vi "Test_pgADONet_dist.vi"() -> ()   [LabVIEW 2026]
uses:
  <vilib>/Viviota/shared/ORM.lvlibp/TypeMap/TypeMap.lvclass
  <vilib>/Viviota/shared/ORM_lib.lvlibp/ObjectRow/ObjectLUT.lvclass
  <vilib>/numeric/Random Number (Range) I64.vi
  <vilib>/numeric/Random Number (Range) DBL.vi
  f3693442-7653-4e44-a421-498bef5f0c13.vi
  <vilib>/Analysis/baseanly.llb/Mean (DBL).vi
  <vilib>/numeric/sub_Random U32.vi
  <vilib>/Viviota/shared/ORM_ADONet.lvlibp/ADOMapper/ADOMapper.lvclass
  C:/Program Files/National Instruments/LabVIEW 2026/vi.lib/Viviota/shared/ORM.lvlibp/SqlMapper/SqlMapper.lvclass
  <vilib>/JDP Science/JSONtext/Variant to JSON Text.vi
  <vilib>/Viviota/shared/ORM_lib.lvlibp/ObjectRow/Write LUT.vi
  <vilib>/Viviota/shared/ORM_DBC_Npgsql_netCore.lvlibp/Postgresql Connect.vi
  <vilib>/Viviota/shared/ORM_pgsql_jdp.lvlibp/dbc/Postgresql Connect.vi
  <vilib>/Viviota/shared/ORM_DBC_Npgsql.lvlibp/Postgresql Connect.vi
  <vilib>/Viviota/shared/ORM.lvlibp/SqlMapper/Read DbConnection.vi
  <vilib>/Viviota/shared/ORM.lvlibp/DbConnection/Write SupportTX.vi
  <vilib>/Viviota/shared/ORM.lvlibp/SqlMapper/Write DbConnection.vi
  <vilib>/Viviota/shared/ORM.lvlibp/TypeMap/Write Table Name.vi
  <vilib>/Viviota/shared/ORM.lvlibp/TypeMap/Write Autokey.vi
  <vilib>/Viviota/shared/ORM_lib.lvlibp/ObjectRow/Read LUT.vi
  <vilib>/JDP Science/JSONtext/LVClass Serializer/JSONtext LVClass Serializer.lvclass
  <vilib>/Viviota/shared/ORM_ADONetCore.lvlibp/ADOMapper/ADOMapper.lvclass
  <vilib>/Viviota/shared/ORM.lvlibp/DbConnection/DbConnection.lvclass
  <vilib>/Viviota/shared/ORM.lvlibp/SqlMapper/SqlMapper.lvclass
  C:/Program Files/National Instruments/LabVIEW 2026/vi.lib/Viviota/shared/ORM_ADONetCore.lvlibp/ADOMapper/ADOMapper.lvclass
  C:/Program Files/National Instruments/LabVIEW 2026/vi.lib/Viviota/shared/ORM_ADONet.lvlibp/ADOMapper/ADOMapper.lvclass
  <vilib>/Analysis/NI_AALBase.lvlib
  <vilib>/Viviota/Viviota ORM - NetCore Connections/dotNetCore/NetCore_API/ORM_API_NetCore.lvlib
  <vilib>/Viviota/Viviota ORM - Direct Connections/DirectConnections/API/ORM_API_jdp.lvlib
  <vilib>/Viviota/Viviota ORM/ORM_API/ORM_API.lvlib
  <vilib>/Viviota/shared/ORM_DBC_Npgsql_netCore.lvlibp/DBC.lvclass
  <vilib>/Viviota/shared/ORM_pgsql_jdp.lvlibp/dbc/DBC.lvclass
  <vilib>/Viviota/shared/ORM_DBC_Npgsql.lvlibp/DBC.lvclass
panel:
  out "Numeric 2":i32
  out "Numeric":i32
  out "mean 3":dbl format="%0.6f"
  out "mean 2":dbl format="%0.6f"
  out "mean":dbl format="%0.6f"
  out "x-y":dbl[](array[numeric])
  out "Array 2":dbl[](array[numeric])
  out "Array":dbl[](array[numeric])
  out "LUT 2":variant[](array[variant])
  out "LUT":variant[](array[variant])
  out "id":i32[](array[numeric])
  # "0.016\n0.084\n0.040"
  # "0.0171\n0.00513\n0.00119"
  # "0.0187\n0.0159\n0.0041"
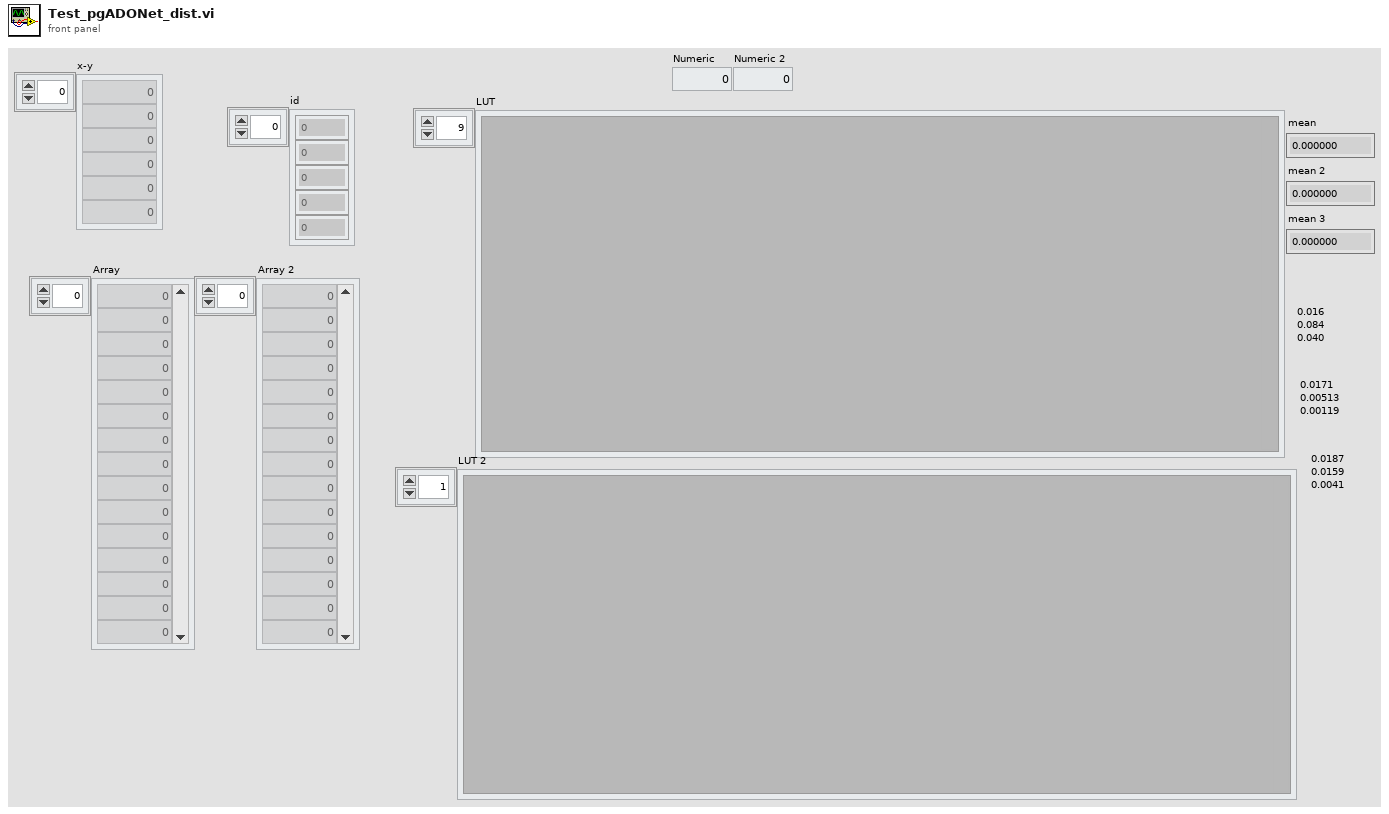
[diagram p1: front panel]
types:
  T1 = cluster{"Text":string, "Integer":i32, "dbl":dbl, "timestamp":timestamp}
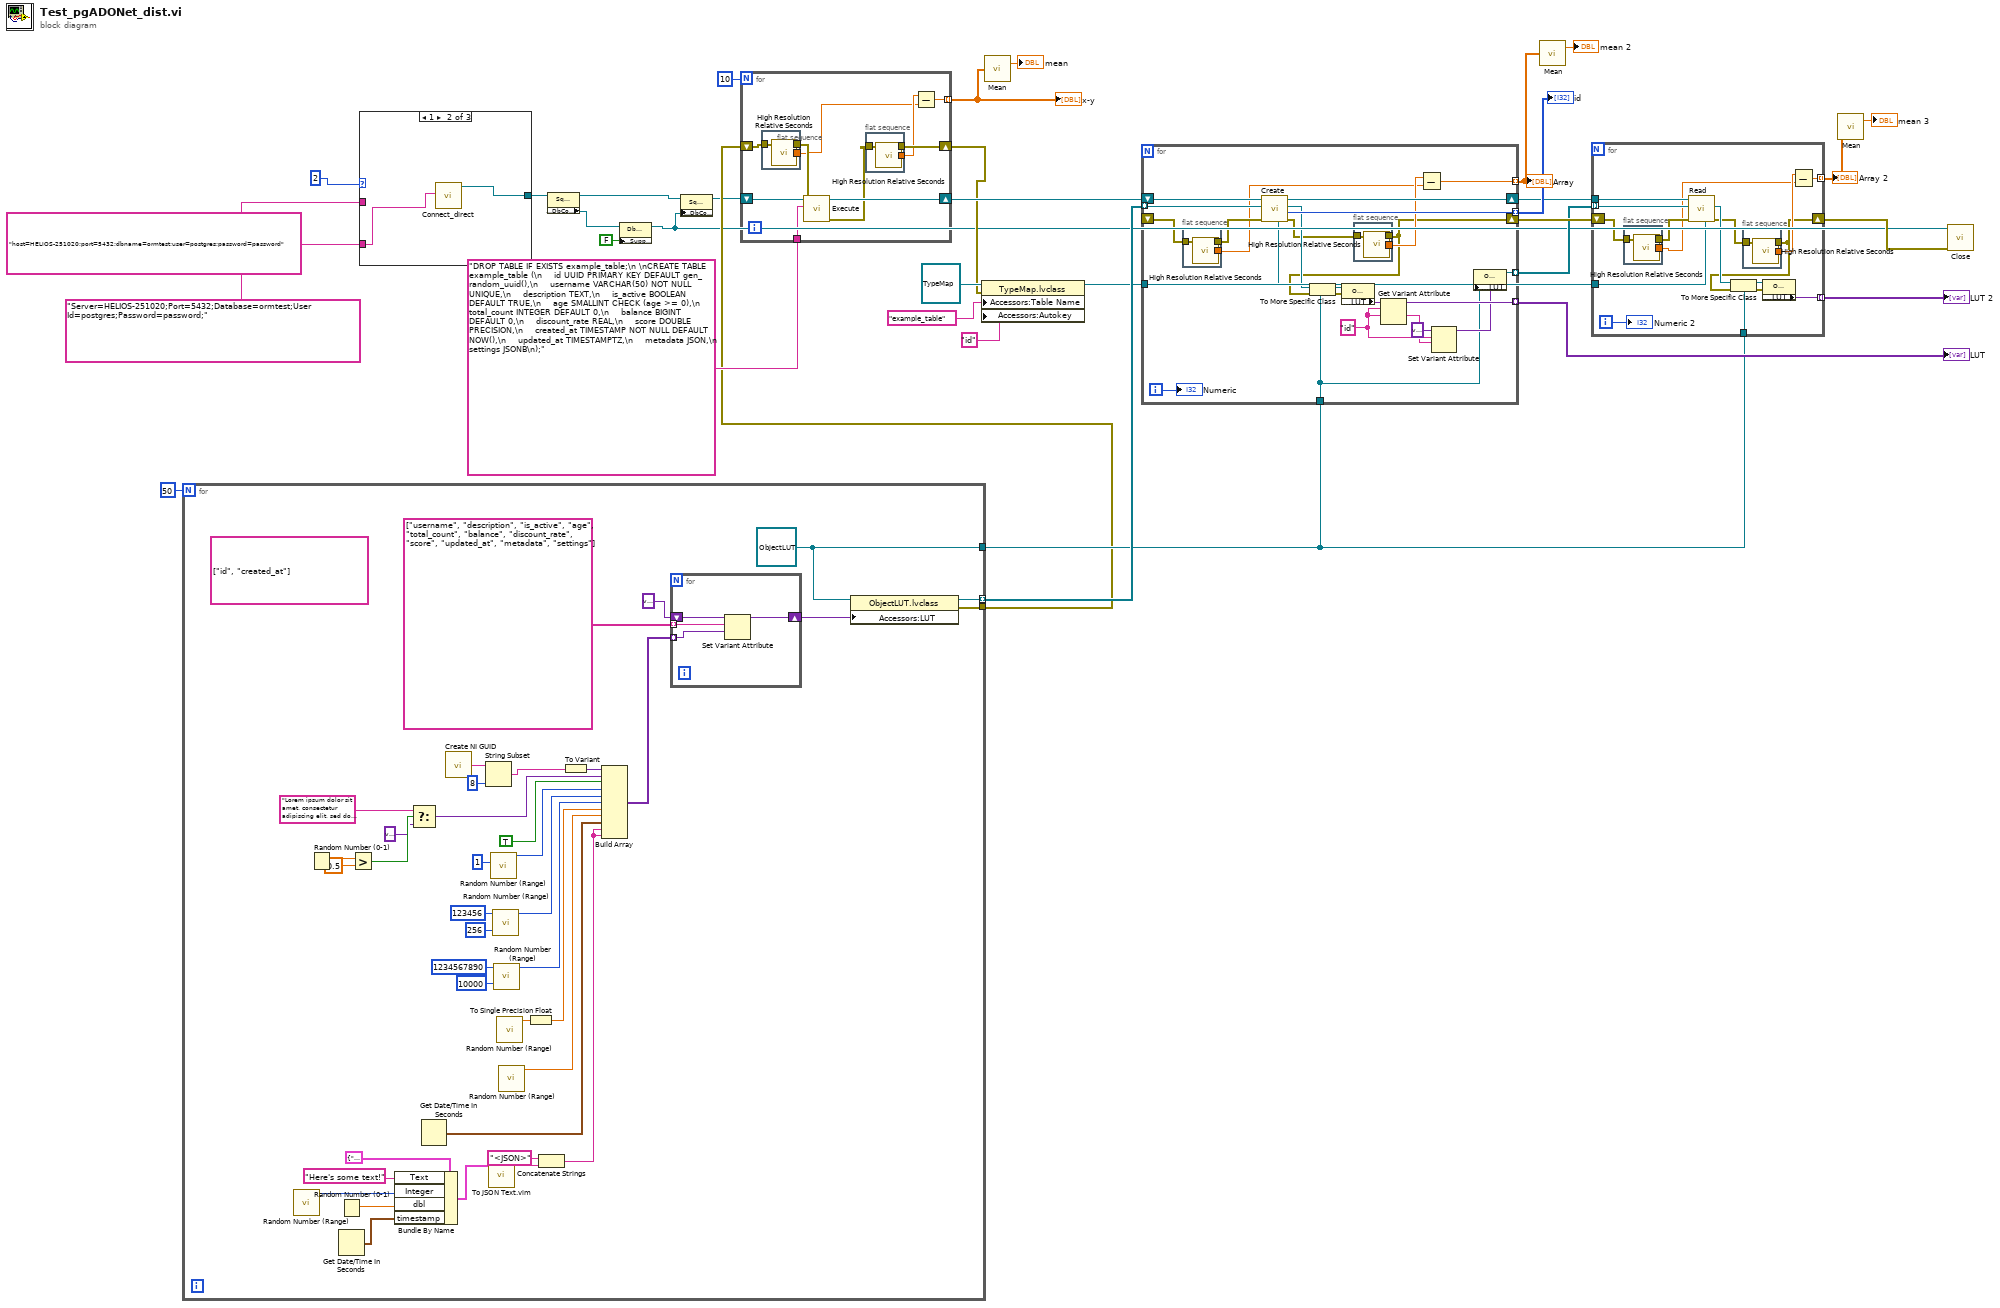
[diagram p0: block diagram]
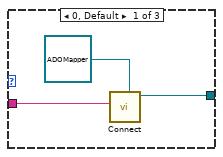
[diagram p2: hidden frame]
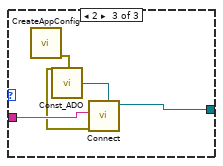
[diagram p3: hidden frame]
diagram:
  n1 = for {
    N: 50 -> [_]
    tunnel: [w41] -> w33 mode=indexing
    tunnel: [w40] -> w23
    tunnel: [w35] -> w18
    w40 = refnum<class "ObjectLUT.lvclass"> refnum ("ORM_lib.lvlibp:ObjectLUT.lvclass")
    (unwired) string[] ["id", "created_at"]
    n2 = call-poly <vilib>:"Random Number (Range).vi"() -> ("number"=w48:i64)  [unwired: 11 in]
    n3 = Random Number (0-1)() -> (number: 0 to 1=w57:dbl)
    n4 = Random Number (0-1)() -> (number: 0 to 1=w49:dbl)
    n5 = Get Date/Time In Seconds() -> (seconds since 1Jan1904=w50:timestamp)
    n6 = Greater?(x=w57, y=0.5) -> (0:w55:bool)
    n7 = Bundle By Name(cluster=T1 {"Text"="This is a test", "Integer"=0, "dbl"=0.0, "timestamp"=timestamp(0 s since 1904-01-01)}, "Text"="Here's some text!", "Integer"=w48, "dbl"=w49, "timestamp"=w50) -> (w46:T1)
    n8 = Select(t="Lorem ipsum dolor sit amet, consectetur adipiscing elit, sed do eiusmod tempor incididunt ut labore et dolore magna aliqua", s=w55, f=variant) -> (s? t:f=w53:variant)
    n9 = Get Date/Time In Seconds() -> (seconds since 1Jan1904=w47:timestamp)
    n10 = call <vilib>:"Create NI GUID.vi"() -> ("NI GUID"=w73:string)
    n11 = String Subset(string=w73, length (rest)=8 ("length (rest)")) -> (substring=w68:string)  [unwired: 1 in]
    n12 = call "To JSON Text.vim"("Anything"=w46) -> ("<JSON>"=w39:string)  [unwired: 9 in, 1 out]
    n13 = call-poly <vilib>:"Random Number (Range).vi"("lower bound (-100)"=i64 1) -> ("number"=w65:i64)  [unwired: 10 in]
    n14 = call-poly <vilib>:"Random Number (Range).vi"("lower bound (-100)"=i64 256, "upper bound (100)"=i64 123456) -> ("number"=w64:i64)  [unwired: 9 in]
    n15 = call-poly <vilib>:"Random Number (Range).vi"("lower bound (-100)"=i64 10000, "upper bound (100)"=i64 1234567890) -> ("number"=w63:i64)  [unwired: 9 in]
    n16 = call-poly <vilib>:"Random Number (Range).vi"() -> ("number"=w61:dbl)  [unwired: 11 in]
    n17 = call-poly <vilib>:"Random Number (Range).vi"() -> ("number"=w59:dbl)  [unwired: 11 in]
    n18 = To Single Precision Float(number=w61) -> (single precision float=w60:sgl)
    n19 = Concatenate Strings("<JSON>" ("string"), w39) -> (w38:string)
    n20 = To Variant(anything=w68) -> (Variant=w67:variant)
    n21 = Build Array(w67, w53, TRUE, w65, w64, w63, w60, w59, w47, w38, w38) -> (w44:variant[])
    n22 = for {
      tunnel: string[] ["username", "description", "is_active", "age", "total_count", "balance", "discount_rate", "score", "updated_at", "metadata", "settings"] -> [w77] mode=indexing
      tunnel: w44 -> [w76] mode=indexing
      shift-right: [w75] -> w42
      shift-left: variant -> [w74]
      n23 = Set Variant Attribute(Variant=w74, name=w77, value=w76) -> (Variant out=w75:variant)  [unwired: 1 in, 2 out]
    }
    n24 = property class="ObjectLUT.lvclass"(reference=w40, "Accessors:LUT"=w42) -> (reference out=w41:refnum<class "ObjectLUT.lvclass">, error out=w35:errorcluster)  [unwired: 1 in]
  }
  n25 = case shown="1" 2 {
    tunnel: "Server=HELIOS-251020;Port=5432;Database=ormtest;User Id=postgres;Password=password;" ("Connection String") -> [w80 _ w84]
    tunnel: [w78 w82 w86] -> w8
    tunnel: "host=HELIOS-251020;port=5432;dbname=ormtest;user=postgres;password=password" ("Connection String") -> [_ w81 _]
    frame 0, Default {
      n26 = call-poly <vilib>:"Connect.vi"("SqlMapper Type"=refnum<class "ADOMapper.lvclass"> refnum ("ORM_ADONetCore.lvlibp:ADOMapper.lvclass"), "Connection String"=w80) -> ("SqlMapper out"=w78:refnum<class "ADOMapper.lvclass">)  [unwired: 8 in, 1 out]
    }
    frame 1 {
      n27 = call-poly <vilib>:"Connect_direct.vi"("Connection String"=w81) -> ("SqlMapper out"=w82:refnum<class "SqlMapper.lvclass">)  [unwired: 9 in, 1 out]
    }
    frame 2 {
      n28 = call <vilib>:"CreateAppConfig.vi"() -> ("error out"=w83:errorcluster)  [unwired: 11 in]
      n29 = call <vilib>:"Const_ADO.vi"() -> ("ADOMapper"=w85:refnum<class "ADOMapper.lvclass">)
      n30 = call-poly <vilib>:"Connect.vi"("SqlMapper Type"=w85, "error in (no error)"=w83, "Connection String"=w84) -> ("SqlMapper out"=w86:refnum<class "ADOMapper.lvclass">)  [unwired: 7 in, 1 out]
    }
  }
  n31 = property class="SqlMapper.lvclass"(reference=w8) -> (reference out=w5:refnum<class "SqlMapper.lvclass">, "Accessors:DbConnection"=w7:refnum<class "DbConnection.lvclass">)  [unwired: 1 in, 1 out]
  n32 = property class="DbConnection.lvclass"(reference=w7, "Accessors:SupportTX"=FALSE ("SupportTX")) -> (reference out=w3:refnum<class "DbConnection.lvclass">)  [unwired: 1 in, 1 out]
  n33 = property class="SqlMapper.lvclass"(reference=w5, "Accessors:DbConnection"=w3) -> (reference out=w4:refnum<class "SqlMapper.lvclass">)  [unwired: 1 in, 1 out]
  n34 = for {
    N: 10 -> [_]
    tunnel: "DROP TABLE IF EXISTS example_table;\n \nCREATE TABLE example_table (\n    id UUID PRIMARY KEY DEFAULT gen_random_uuid(),\n    username VARCHAR(50) NOT NULL UNIQUE,\n    description TEXT,\n    is_active BOOLEAN DEFAULT TRUE,\n    age SMALLINT CHECK (age >= 0),\n    total_count INTEGER DEFAULT 0,\n    balance BIGINT DEFAULT 0,\n    discount_rate REAL,\n    score DOUBLE PRECISION,\n    created_at TIMESTAMP NOT NULL DEFAULT NOW(),\n    updated_at TIMESTAMPTZ,\n    metadata JSON,\n    settings JSONB\n);" ("sql") -> [w95]
    tunnel: [w87] -> w14 mode=indexing
    shift-right: [w94] -> w25
    shift-left: w4 -> [w96]
    shift-right: [w90] -> w17
    shift-left: w18 -> [w93]
    n35 = flat-sequence {
      tunnel: [w100] -> w88
      tunnel: w93 -> [w99]
      tunnel: [w99] -> w92
      frame #0 {
        n36 = call <vilib>:"High Resolution Relative Seconds.vi"() -> ("relative seconds"=w100:dbl)
      }
    }
    n37 = call-dynamic "Execute.vi"("error in (no error)"=w92, "sql"=w95, "SqlMapper in"=w96) -> ("error out"=w91:errorcluster, "SqlMapper out"=w94:refnum<class "SqlMapper.lvclass">)  [unwired: 6 in, 1 out]
    n38 = flat-sequence {
      tunnel: [w98] -> w89
      tunnel: w91 -> [w97]
      tunnel: [w97] -> w90
      frame #0 {
        n39 = call <vilib>:"High Resolution Relative Seconds.vi"() -> ("relative seconds"=w98:dbl)
      }
    }
    n40 = Subtract(x=w89, y=w88) -> (x-y=w87:dbl)
  }
  "x-y" <- w14
  n41 = property class="TypeMap.lvclass"(reference=refnum<class "TypeMap.lvclass"> refnum ("TypeMap in"), error in=w17, "Accessors:Table Name"="example_table" ("Table Name"), "Accessors:Autokey"="id" ("Autokey")) -> (reference out=w24:refnum<class "TypeMap.lvclass">)  [unwired: 1 out]
  n42 = call-poly <vilib>:"Mean.vi"("X"=w14) -> ("mean"=→"mean":dbl)  [unwired: 1 out]
  n43 = for {
    tunnel: w33 -> [w123] mode=indexing
    tunnel: w24 -> [w122]
    tunnel: [w121] -> w30 mode=indexing
    tunnel: w23 -> [w111]
    tunnel: [w116] -> w29 mode=indexing
    shift-right: [w102] -> w27
    shift-left: _ -> [w109]
    tunnel: [w110] -> w26 mode=indexing
    shift-right: [w106] -> w19
    shift-left: w25 -> [w124]
    tunnel: [w103] -> w11 mode=indexing
    i -> [w101]
    w114 = "id" ("name")
    n44 = flat-sequence {
      tunnel: [w128] -> w104
      tunnel: w109 -> [w127]
      tunnel: [w127] -> w108
      frame #0 {
        n45 = call <vilib>:"High Resolution Relative Seconds.vi"() -> ("relative seconds"=w128:dbl)
      }
    }
    n46 = call-dynamic "Create.vi"("TypeMap in"=w122, "error in (no error)"=w108, "object in"=w123, "SqlMapper in"=w124) -> ("error out"=w107:errorcluster, "id"=w121:i32, "object out"=w120:refnum<class>, "SqlMapper out"=w106:refnum<class "SqlMapper.lvclass">)  [unwired: 4 in]
    n47 = To More Specific Class(target class=w111, reference=w120, error in=w102) -> (specific class reference=w118:refnum<class "ObjectLUT.lvclass">, error out=w119:errorcluster)
    n48 = property class="ObjectLUT.lvclass"(reference=w118, error in=w119) -> ("Accessors:LUT"=w117:variant)  [unwired: 2 out]
    n49 = flat-sequence {
      tunnel: [w126] -> w105
      tunnel: w107 -> [w125]
      tunnel: [w125] -> w102
      frame #0 {
        n50 = call <vilib>:"High Resolution Relative Seconds.vi"() -> ("relative seconds"=w126:dbl)
      }
    }
    n51 = Get Variant Attribute(Variant=w117, name=w114, default value (empty Variant)=w114) -> (duplicate Variant=w116:variant, value=w113:string)  [unwired: 1 in, 2 out]
    n52 = Subtract(x=w105, y=w104) -> (x-y=w103:dbl)
    n53 = Set Variant Attribute(Variant=variant ("variant"), name=w114, value=w113) -> (Variant out=w112:variant)  [unwired: 1 in, 2 out]
    n54 = property class="ObjectLUT.lvclass"(reference=w111, "Accessors:LUT"=w112) -> (reference out=w110:refnum<class "ObjectLUT.lvclass">)  [unwired: 1 in, 1 out]
    "Numeric" <- w101
  }
  "id" <- w30
  "LUT" <- w29
  "Array" <- w11
  n55 = call-poly <vilib>:"Mean.vi"("X"=w11) -> ("mean"=→"mean 2":dbl)  [unwired: 1 out]
  n56 = for {
    tunnel: w26 -> [w144] mode=indexing
    tunnel: w19 -> [w143]
    tunnel: w24 -> [w142]
    tunnel: w23 -> [w138]
    tunnel: [w137] -> w22 mode=indexing
    shift-right: [w130] -> w21
    shift-left: w27 -> [w136]
    tunnel: [w131] -> w10 mode=indexing
    i -> [w129]
    n57 = flat-sequence {
      tunnel: [w148] -> w132
      tunnel: w136 -> [w147]
      tunnel: [w147] -> w135
      frame #0 {
        n58 = call <vilib>:"High Resolution Relative Seconds.vi"() -> ("relative seconds"=w148:dbl)
      }
    }
    n59 = call-dynamic "Read.vi"("TypeMap in"=w142, "error in (no error)"=w135, "object in"=w144, "SqlMapper in"=w143) -> ("error out"=w134:errorcluster, "Value"=w139:refnum<class>)  [unwired: 4 in, 2 out]
    n60 = To More Specific Class(target class=w138, reference=w139, error in=w130) -> (specific class reference=w141:refnum<class "ObjectLUT.lvclass">, error out=w140:errorcluster)
    n61 = flat-sequence {
      tunnel: [w146] -> w133
      tunnel: w134 -> [w145]
      tunnel: [w145] -> w130
      frame #0 {
        n62 = call <vilib>:"High Resolution Relative Seconds.vi"() -> ("relative seconds"=w146:dbl)
      }
    }
    n63 = property class="ObjectLUT.lvclass"(reference=w141, error in=w140) -> ("Accessors:LUT"=w137:variant)  [unwired: 2 out]
    n64 = Subtract(x=w133, y=w132) -> (x-y=w131:dbl)
    "Numeric 2" <- w129
  }
  "LUT 2" <- w22
  "Array 2" <- w10
  n65 = call-poly <vilib>:"Mean.vi"("X"=w10) -> ("mean"=→"mean 3":dbl)  [unwired: 1 out]
  n66 = call-dynamic "Close.vi"("error in (no error)"=w21, "DbConnection in"=w3) -> ()  [unwired: 9 in, 1 out]
